vi "VIH Constant - Default Edit Programs Association.vi"() -> (3 "Default Edit Programs":T1(array[cluster]))   [LabVIEW 2014]
doc: "::: VI Helpeks :::\nCopyright (c) 2000-2026 Konstantin Shifershteyn. All rights reserved."
panel:
  # "VI Helpeks\nCopyright (c) 2012-2026 Konstantin Shifershteyn"
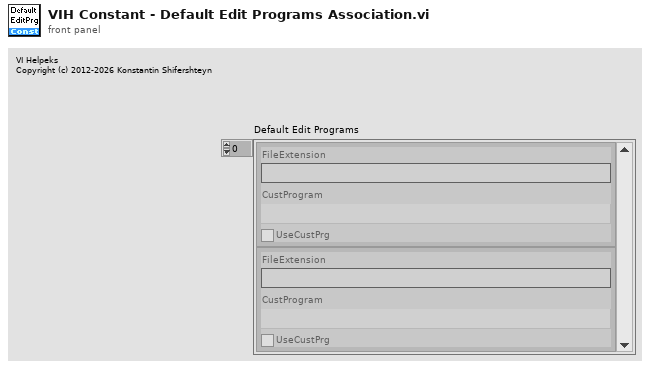
[diagram p1: front panel]
types:
  T1 = cluster{"FileExtension":string, "CustProgram":path, "UseCustPrg":bool}[]
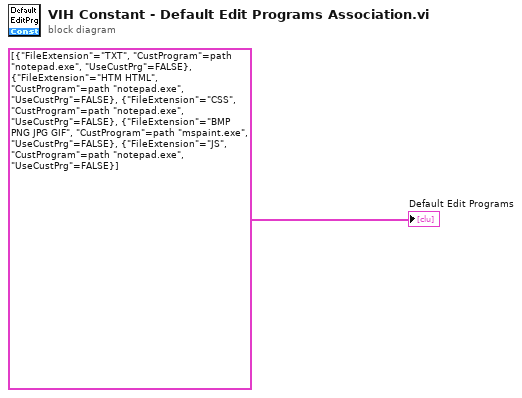
[diagram p0: block diagram]
diagram:
  "Default Edit Programs" <- T1 [{"FileExtension"="TXT", "CustProgram"=path "notepad.exe", "UseCustPrg"=FALSE}, {"FileExtension"="HTM HTML", "CustProgram"=path "notepad.exe", "UseCustPrg"=FALSE}, {"FileExtension"="CSS", "CustProgram"=path "notepad.exe", "UseCustPrg"=FALSE}, {"FileExtension"="BMP PNG JPG GIF", "CustProgram"=path "mspaint.exe", "UseCustPrg"=FALSE}, {"FileExtension"="JS", "CustProgram"=path "notepad.exe", "UseCustPrg"=FALSE}] ("EditPrgs")
